vi "ZM-ROOT-init.vi"(8 "error in":errorcluster, 11 "ZM-ROOT-root in":refnum<class "ZM-ROOT-root.lvclass">) -> (0 "error out":errorcluster, 2 "Event Registration Refnum":refnum<event-registration>, 3 "ZM-ROOT-root out":refnum<class "ZM-ROOT-root.lvclass">)   [LabVIEW 2020, in "ZM-ROOT-root.lvlib" / "ZM-ROOT-root.lvclass"]
doc: "Init of the root, run in Actor Core before Call Parent: launches the CM, then the HWM, and registers for the stop and error user events, handing the registration to ZM-ROOT-helperPanel. Registering before the actor runs means a stop is never lost. A launch or registration error goes on into Call Parent, so the root stops at once."
uses:
  ZM-ROOT-root.lvclass
  ZM-ROOT-root.lvclass/ZM-ROOT-root.ctl
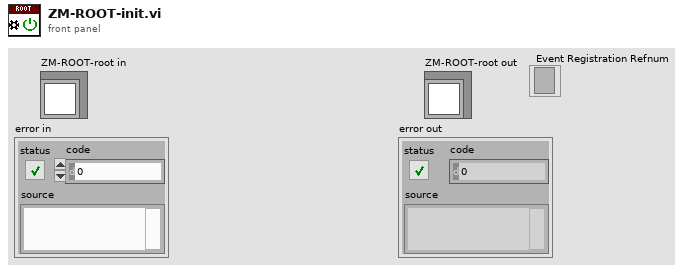
[diagram p1: front panel]
types:
  T1 = typedef "ZM-ROOT-root.lvlib/ZM-ROOT-root.lvclass/ZM-ROOT-EVENTS.ctl" = cluster{"stop":refnum<user-event>, "error":refnum<user-event>}
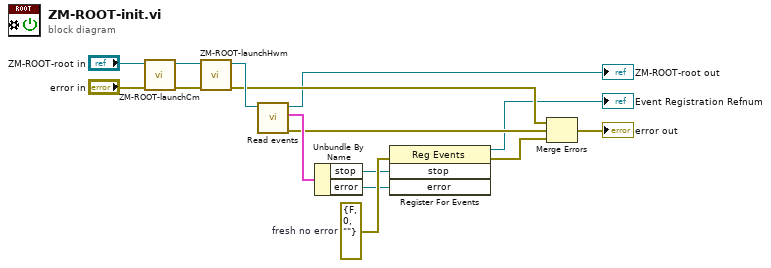
[diagram p0: block diagram]
diagram:
  w9 = errorcluster {"status"=FALSE, "code"=0, "source"=""}  # fresh no error
  n1 = call "ZM-ROOT-launchCm.vi"("error in (no error)"="error in", "ZM-ROOT-root in"="ZM-ROOT-root in") -> ("error out"=w13:errorcluster, "ZM-ROOT-root out"=w12:refnum<class "ZM-ROOT-root.lvclass">)  [unwired: 8 in]
  n2 = call "ZM-ROOT-launchHwm.vi"("error in (no error)"=w13, "ZM-ROOT-root in"=w12) -> ("error out"=w6:errorcluster, "ZM-ROOT-root out"=w11:refnum<class "ZM-ROOT-root.lvclass">)  [unwired: 8 in]
  n3 = call "Read events.vi"("ZM-ROOT-root in"=w11) -> ("error out"=w5:errorcluster, "ZM-ROOT-EVENTS"=w10:T1, "ZM-ROOT-root out"=→"ZM-ROOT-root out":refnum<class "ZM-ROOT-root.lvclass">)  [unwired: 8 in]
  n4 = Unbundle By Name(w10) -> ("stop"=w8:refnum<user-event>, "error"=w7:refnum<user-event>)
  n5 = register-events(error in=w9, w8, w7) -> (reference out=→"Event Registration Refnum":refnum<event-registration>, error out=w4:errorcluster)  [unwired: 1 in]
  n6 = Merge Errors(w6, w5, w4) -> (→"error out":errorcluster)
